vi "Game_Loop.vi"(0 "Channels":T3, 5 "State":T2={"Tick"=0, "Phase"=0, "PhaseTicks"=0, "Level"=1, "Room"=0, "X10"=0, "Y10"=0, "VY10"=0, "Mode"=0, "Facing"=0, "Run"=0, "Vert"=0, "StandY"=0, "EntryX10"=0, "EntryY10"=0, "EntryMode"=0, "Lives"=4, "Score"=0, "NextLife"=10000, "KeyR"=0, "KeyB"=0, "KeyY"=0, "Torch"=FALSE, "FloorPhase"=0, "Dead"=FALSE, "LevelStart"=FALSE, "Quit"=FALSE, "Sound"=0, "Seed"=12345, "DemoStep"=0, "Tiles"=[], "World"=[], "Enemies"=[], "Highscores"=[], "Name"=[0, 0, 0], "Cursor"=0}, 7 "Rooms":T1(array[cluster]), 11 "error in":errorcluster) -> (4 "Cheat used":bool, 15 "error out":errorcluster)   [LabVIEW 2020, in "GH_App.lvlib"]
doc: "The game loop of Main as a subVI, so that it runs in its own execution system (standard) and never needs the user interface thread: Engine_Tick 60 times per second, paced by Frame_Pace, until Stop. Timing log: the start time of every tick (ms) and the game tick, the last 3600 ticks, written to Resourcesòta\\timing_game.csv at the end (Timing_Save) - only when the cheat mode was on at some point (Cheat used, also for the picture log of Main)."
uses:
  GH_App.lvlib
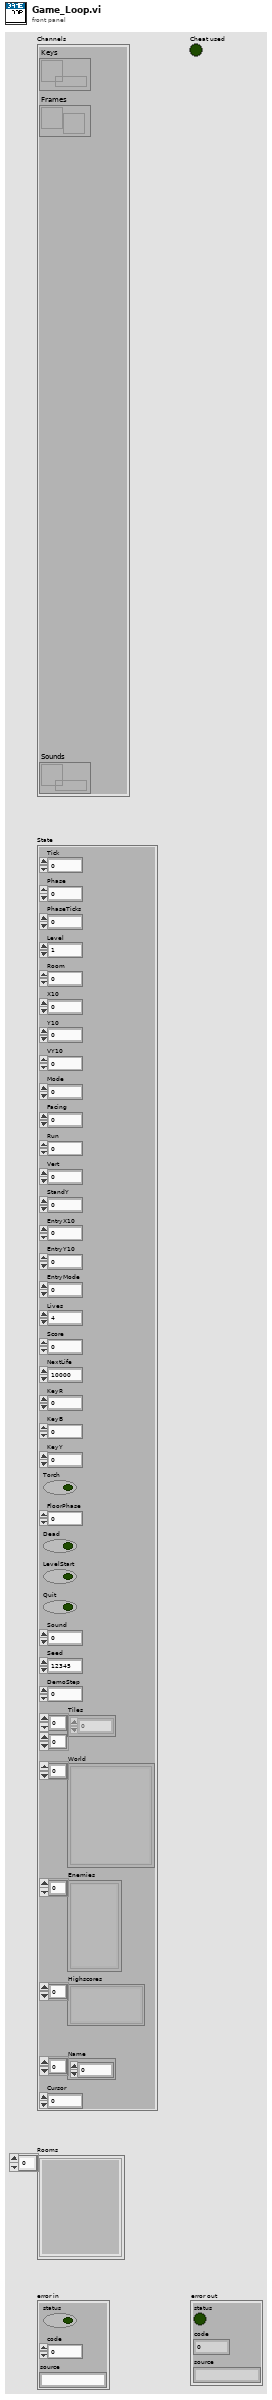
[diagram p1: front panel]
types:
  T1 = cluster{"ID":string, "Depth":i32, "Column":i32, "Tiles":u8[][]}[]
  T2 = cluster{"Tick":u32, "Phase":i32, "PhaseTicks":i32, "Level":i32, "Room":i32, "X10":i32, "Y10":i32, "VY10":i32, "Mode":i32, "Facing":i32, "Run":i32, "Vert":i32, "StandY":i32, "EntryX10":i32, "EntryY10":i32, "EntryMode":i32, "Lives":i32, "Score":i32, "NextLife":i32, "KeyR":i32, "KeyB":i32, "KeyY":i32, "Torch":bool, "FloorPhase":i32, "Dead":bool, "LevelStart":bool, "Quit":bool, "Sound":i32, "Seed":u32, "DemoStep":i32, "Tiles":u8[][], "World":cluster{"ID":string, "Depth":i32, "Column":i32, "Tiles":u8[][]}[], "Enemies":cluster{"Kind":i32, "X10":i32, "Y10":i32, "Dir":i32, "Mode":i32}[], "Highscores":cluster{"Score":i32, "Name":string}[], "Name":i32[], "Cursor":i32}
  T3 = cluster{"Keys":refnum<queue>, "Frames":refnum<notifier>, "Sounds":refnum<queue>}
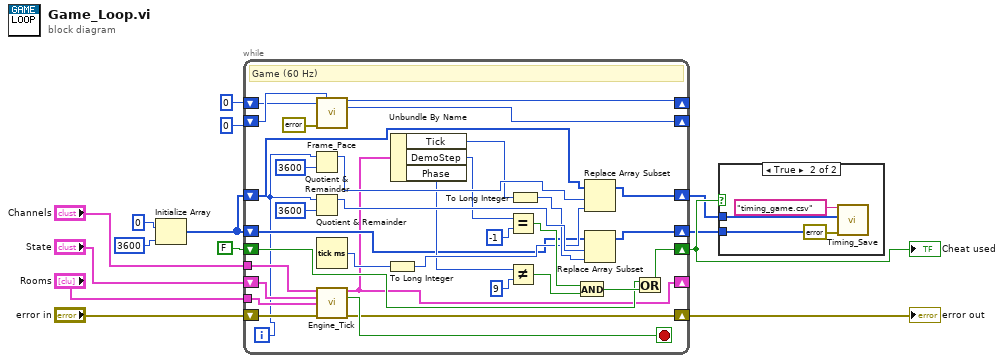
[diagram p0: block diagram]
diagram:
  n1 = Initialize Array(0, 3600) -> (w7:i32[])
  n2 = while {
    tunnel: "Channels" -> [w16]
    tunnel: "Rooms" -> [w17]
    shift-right: [w19] -> _
    shift-left: "State" -> [w18]
    shift-right: [w21] -> w11
    shift-left: "error in" -> [w20]
    shift-right: [w23] -> _
    shift-left: u32 0 ("Start ms") -> [w22]
    shift-right: [w25] -> _
    shift-left: 0 -> [w24]
    shift-right: [w31] -> w14
    shift-left: FALSE ("no cheat yet") -> [w30]
    shift-right: [w27] -> w12
    shift-left: w7 -> [w26]
    shift-right: [w29] -> w13
    shift-left: w7 -> [w28]
    i -> [w15]
    stop <- w33 stop-if-true
    # "Game (60 Hz)"
    n3 = Quotient & Remainder(x=w15, y=3600) -> (x-y*floor(x/y)=w40:i32)  [unwired: 1 out]
    n4 = Quotient & Remainder(x=w15, y=3600) -> (x-y*floor(x/y)=w43:i32)  [unwired: 1 out]
    n5 = call "Frame_Pace.vi"("Start ms"=w22, "Count"=w24, "error in"=errorcluster {"status"=FALSE, "code"=0, "source"=""} ("no error")) -> ("Start out"=w23:u32, "Count out"=w25:i32)  [unwired: 10 in, 1 out]
    n6 = Tick Count (ms)() -> (millisecond timer value=w32:u32)
    n7 = call "Engine_Tick.vi"("Channels"=w16, "State"=w18, "Rooms"=w17, "error in"=w20) -> ("State out"=w19:T2, "Stop"=w33:bool, "error out"=w21:errorcluster)  [unwired: 9 in]
    n8 = To Long Integer(number=w32) -> (32bit integer=w38:i32)
    n9 = Unbundle By Name(w19) -> ("Tick"=w35:u32, "DemoStep"=w36:i32, "Phase"=w37:i32)
    n10 = Equal?(x=w36, y=-1) -> (x = y?=w45:bool)
    n11 = Not Equal?(x=w37, y=9) -> (x != y?=w47:bool)
    n12 = To Long Integer(number=w35) -> (32bit integer=w41:i32)
    n13 = And(x=w45, y=w47) -> (x .and. y?=w48:bool)
    n14 = Replace Array Subset(array=w26, new element=w38, index=w40) -> (w27:i32[])
    n15 = Replace Array Subset(array=w28, new element=w41, index=w43) -> (w29:i32[])
    n16 = Or(x=w30, y=w48) -> (x .or. y?=w31:bool)
  }
  "Cheat used" <- w14
  "error out" <- w11
  n17 = case shown="True" w14 {
    tunnel: w12 -> [_ w49]
    tunnel: w13 -> [_ w50]
    frame False {
    }
    frame True {
      n18 = call "Timing_Save.vi"("File name"="timing_game.csv", "Ms"=w49, "Tick"=w50, "error in"=errorcluster {"status"=FALSE, "code"=0, "source"=""} ("no error")) -> ()  [unwired: 11 in, 1 out]
    }
  }
